vi "RDC-Lin-Find_tau.vi"(11 "Short Probe reading":T1={"Frequency"=array[2001 elements], "Reflection'"=array[2001 elements], "Reflection''"=array[2001 elements], "Permativity'"=array[2001 elements], "Permativity''"=array[2001 elements], "Conductivity"=array[2001 elements], "Loss Tangent"=array[2001 elements], "Resistance"=[], "Reactance"=[]}) -> (1 "alt tau":dbl format="%#_6p", 2 "Tau":dbl format="%#_6p")   [LabVIEW 2020, in "RDC-Reflection_Data_Computation.lvlib"]
doc: "Finds the delay Tau from the phase of the reflection of a short-probe Common Format cluster by unwrapping and fitting it. Also returns an alternative value, alt tau."
uses:
  RDC-Reflection_Data_Computation.lvlib
  Reflector/RFH-common_data_format.ctl
  <vilib>/Analysis/6fits.llb/Curve Fitting Criteria.ctl
  <vilib>/Analysis/NI_AALPro.lvlib
  Reflector/RFH-Reflection_File_Handler.lvlib
panel:
  out "Linearization of the angle":dbl[][](graph)
  out "Angle allignment":dbl[][](graph)
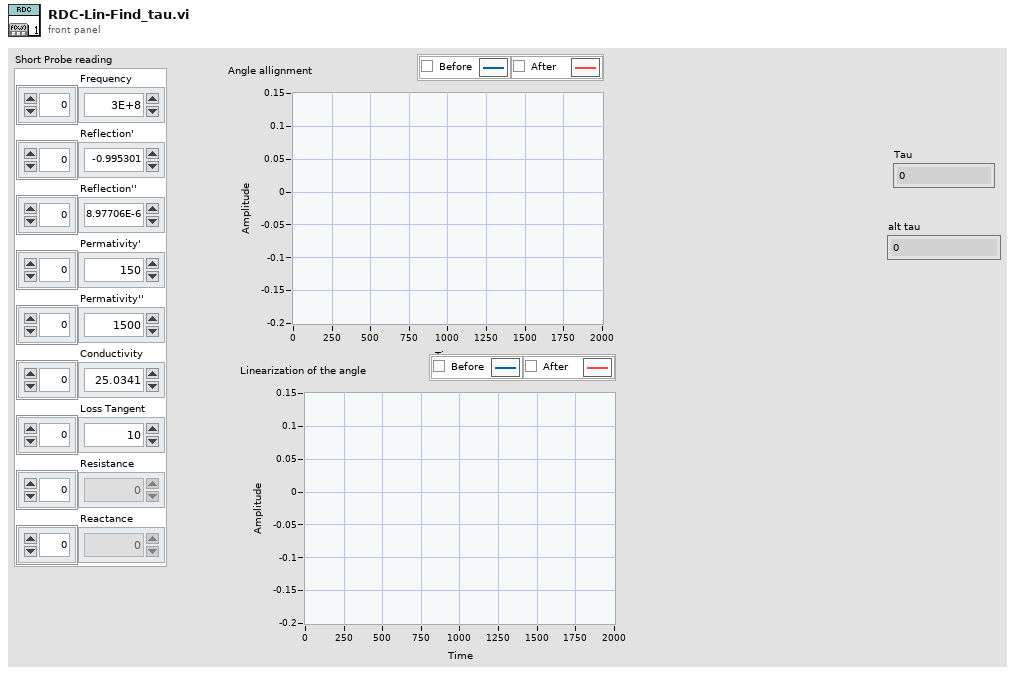
[diagram p1: front panel]
types:
  T1 = typedef "RFH-Reflection_File_Handler.lvlib/RFH-common_data_format.ctl" = cluster{"Frequency":dbl[], "Reflection'":dbl[], "Reflection''":dbl[], "Permativity'":dbl[], "Permativity''":dbl[], "Conductivity":dbl[], "Loss Tangent":dbl[], "Resistance":dbl[], "Reactance":dbl[]}
  T2 = typedef "NI_AALPro.lvlib/Curve Fitting Criteria.ctl" = u16
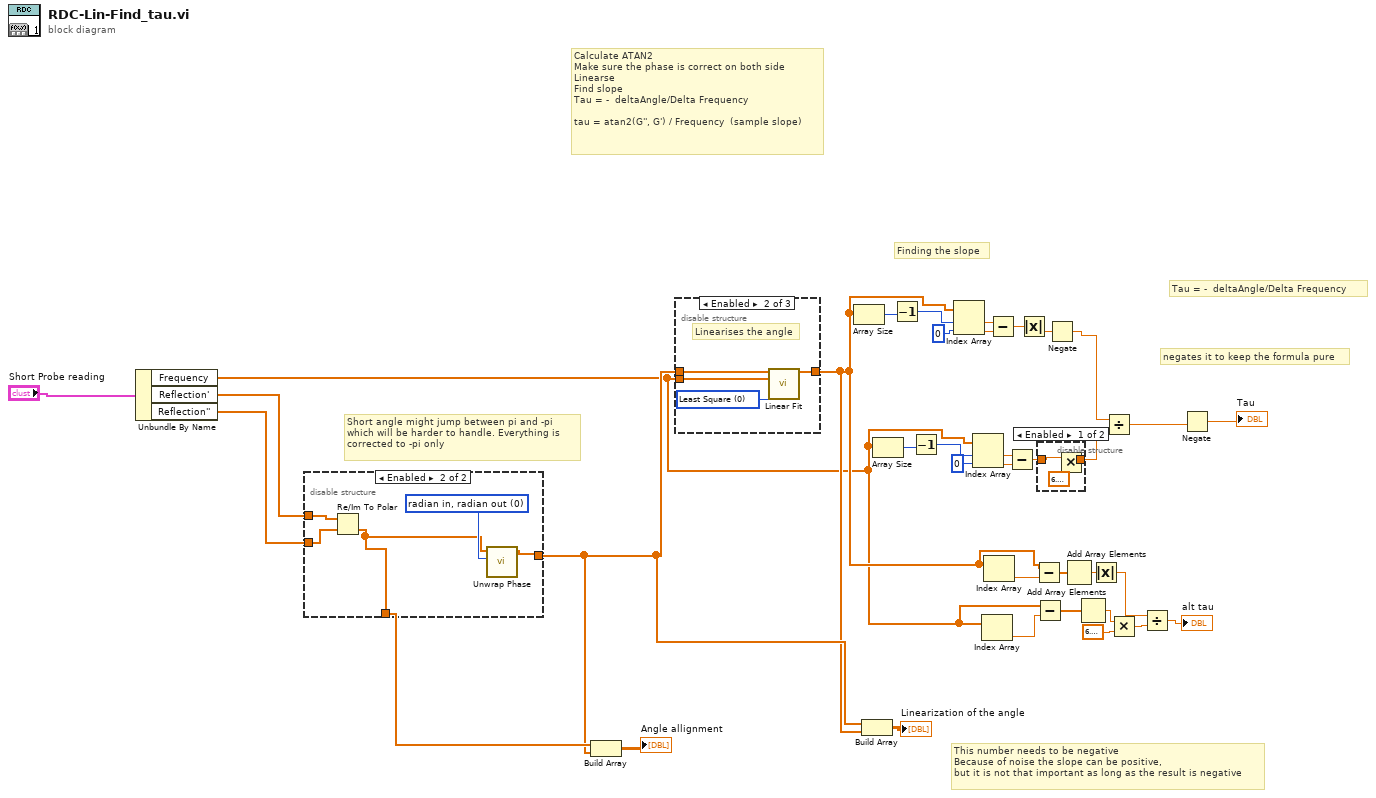
[diagram p0: block diagram]
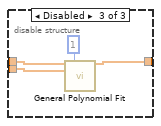
[diagram p4: hidden frame]
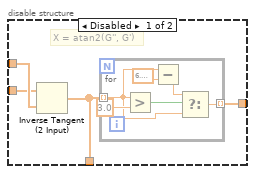
[diagram p5: hidden frame]
diagram:
  # "Calculate ATAN2\nMake sure the phase is correct on both side\nLinearse\nFind slope\nTau = -  deltaAngle/Delta Frequency \n\ntau = atan2(G'', G') / Frequency  (sample slope)"
  # "negates it to keep the formula pure"
  # "Tau = -  deltaAngle/Delta Frequency"
  # "This number needs to be negative\nBecause of noise the slope can be positive,\nbut it is not that important as long as the result is negative"
  # "Finding the slope"
  # "Short angle might jump between pi and -pi\nwhich will be harder to handle. Everything is\ncorrected to -pi only"
  n1 = Unbundle By Name("Short Probe reading") -> ("Frequency"=w6:dbl[], "Reflection'"=w15:dbl[], "Reflection''"=w14:dbl[])
  n2 = disable-structure shown="Enabled" {
    disable-tunnel: [w40 w48] -> w21
    disable-tunnel: [w39 w47] -> w16
    disable-tunnel: w15 -> [w38 w50]
    disable-tunnel: w14 -> [w37 w49]
    frame Disabled {
      # "X = atan2(G'', G')"
      n3 = Inverse Tangent (2 Input)(1:w38, 2:w37) -> (0:w40:dbl[])
      n4 = for {
        tunnel: w40 -> [w42] mode=indexing
        tunnel: [w41] -> w39 mode=indexing
        n5 = Greater?(x=w42, y=3.0) -> (0:w45:bool)
        n6 = Subtract(x=w42, y=6.283185307179586) -> (x-y=w43:dbl)
        n7 = Select(t=w43, s=w45, f=w42) -> (s? t:f=w41:dbl)
      }
    }
    frame Enabled {
      w51 = 0 items=["radian in, radian out", "radian in, degree out", "degree in, degree out", "degree in, radian out"] ("phase unit")
      n8 = Re/Im To Polar(2:w49, 3:w50) -> (0:w48:dbl[])  [unwired: 1 out]
      n9 = call <vilib>:"Unwrap Phase.vi"("phase unit"=w51, "Phase"=w48) -> ("Unwrapped Phase"=w47:dbl[])  [unwired: 8 in, 1 out]
    }
  }
  n10 = Build Array(w21, w16) -> (→"Angle allignment":dbl[][])
  n11 = disable-structure shown="Enabled" {
    disable-tunnel: w6 -> [_ w55 w58]
    disable-tunnel: [w52 w54 w57] -> w10
    disable-tunnel: w16 -> [w52 w53 w59]
    frame Disabled {
    }
    frame Enabled {
      w56 = T2 0 items=["Least Square", "Least Absolute Residual", "Bisquare"] ("method")
      # "Linearises the angle"
      n12 = call <vilib>:"Linear Fit.vi"("Y"=w53, "X"=w55, "method"=w56) -> ("Best Linear Fit"=w54:dbl[])  [unwired: 8 in, 4 out]
    }
    frame Disabled {
      n13 = call <vilib>:"General Polynomial Fit.vi"("Y"=w59, "polynomial order"=1, "X"=w58) -> ("Best Polynomial Fit"=w57:dbl[])  [unwired: 9 in, 3 out]
    }
  }
  n14 = Array Size(array=w10) -> (size(s)=w26:i32)
  n15 = Build Array(w16, w10) -> (→"Linearization of the angle":dbl[][])
  n16 = Array Size(array=w6) -> (size(s)=w35:i32)
  n17 = Decrement(x=w26) -> (x-1=w27:i32)
  n18 = Decrement(x=w35) -> (x-1=w34:i32)
  n19 = Index Array(array=w10, index #1=w27, index #2=0 ("index")) -> (element #1=w29:dbl, element #2=w30:dbl)
  n20 = Index Array(array=w6, index #1=w34, index #2=0 ("index")) -> (element #1=w32:dbl, element #2=w31:dbl)
  n21 = Index Array(array=w6) -> (element=w12:dbl)  [unwired: 1 in]
  n22 = Index Array(array=w10) -> (element=w11:dbl)  [unwired: 1 in]
  n23 = Subtract(x=w29, y=w30) -> (x-y=w24:dbl)
  n24 = Subtract(x=w32, y=w31) -> (x-y=w25:dbl)
  n25 = Absolute Value(x=w24) -> (abs(x)=w19:dbl)
  n26 = Subtract(x=w10, y=w11) -> (x-y=w9:dbl[])
  n27 = Subtract(x=w6, y=w12) -> (x-y=w8:dbl[])
  n28 = disable-structure shown="Enabled" {
    disable-tunnel: w25 -> [w63 w64]
    disable-tunnel: [w62 w64] -> w13
    frame Enabled {
      n29 = Multiply(x=w63, y=6.283185307179586) -> (x*y=w62:dbl)
    }
    frame Disabled {
    }
  }
  n30 = Negate(x=w19) -> (-x=w18:dbl)
  n31 = Add Array Elements(numeric array=w9) -> (sum=w7:dbl)
  n32 = Add Array Elements(numeric array=w8) -> (sum=w3:dbl)
  n33 = Absolute Value(x=w7) -> (abs(x)=w1:dbl)
  n34 = Divide(x=w18, y=w13) -> (x/y=w23:dbl)
  n35 = Multiply(x=w3, y=6.283185307179586) -> (x*y=w2:dbl)
  n36 = Divide(x=w1, y=w2) -> (x/y=→"alt tau":dbl)
  n37 = Negate(x=w23) -> (-x=→"Tau":dbl)
